vi "Update String value.vi"(7 "Interpret as Unicode (T)":bool=TRUE, 8 "error in (no error)":errorcluster, 10 "String Value":string, 11 "String Control Reference In":refnum<vi>) -> (0 "error out":errorcluster, 3 "String Control Reference Out":refnum<vi>)   [LabVIEW 2019, in "Language Selection.lvlib"]
doc: "Uses \"String Value\" to translate String control.\n- - -\nCopyright (c) 2026, Merecs Engineering GmbH"
uses:
  Language Selection.lvlib
panel:
  # "Connector Pane"
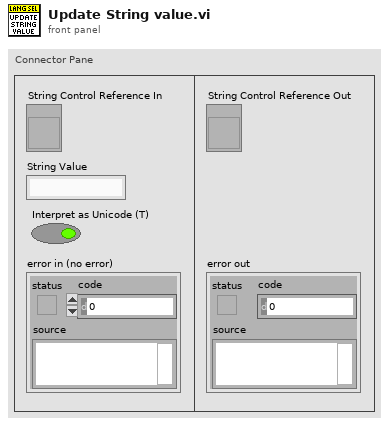
[diagram p1: front panel]
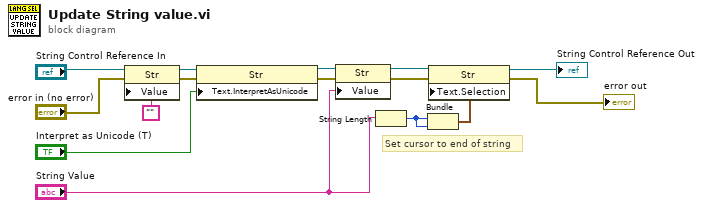
[diagram p0: block diagram]
diagram:
  # "Set cursor to end of string"
  n1 = property class="Str"(reference="String Control Reference In", error in="error in (no error)", "Value"="") -> (reference out=w3:refnum<vi>, error out=w10:errorcluster)
  n2 = property class="Str"(reference=w3, error in=w10, "Text.InterpretAsUnicode"="Interpret as Unicode (T)") -> (reference out=w12:refnum<vi>, error out=w11:errorcluster)
  n3 = property class="Str"(reference=w12, error in=w11, "Value"="String Value") -> (reference out=w4:refnum<vi>, error out=w5:errorcluster)
  n4 = String Length(string="String Value") -> (length=w8:i32)
  n5 = Bundle(w8, w8) -> (w9:cluster{i32, i32})  [unwired: 1 in]
  n6 = property class="Str"(reference=w4, error in=w5, "Text.Selection"=w9) -> (reference out=→"String Control Reference Out":refnum<vi>, error out=→"error out":errorcluster)
